vi "Send Value Update.vi"(8 "error in (no error)":errorcluster, 9 "Value":variant, 10 "Datum Name":string, 11 "IViewModel in":refnum<class "IViewModel.lvclass">) -> (0 "error out":errorcluster)   [LabVIEW 2018, in "MVA Framework.lvlib" / "IViewModel.lvlib" / "IViewModel.lvclass"]
doc: "发送值更新"
uses:
  IViewModel.lvclass
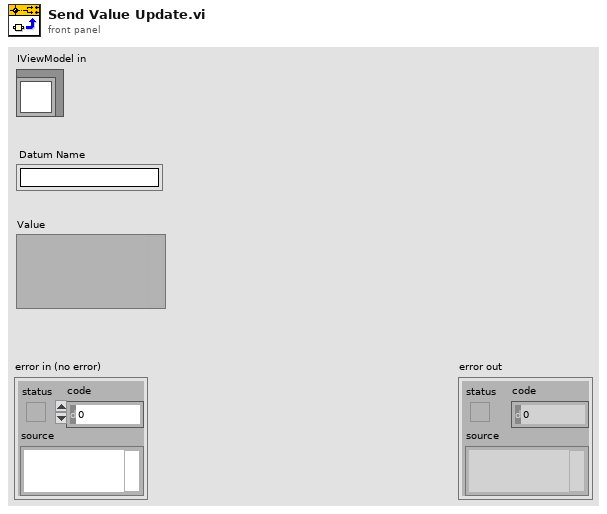
[diagram p1: front panel]
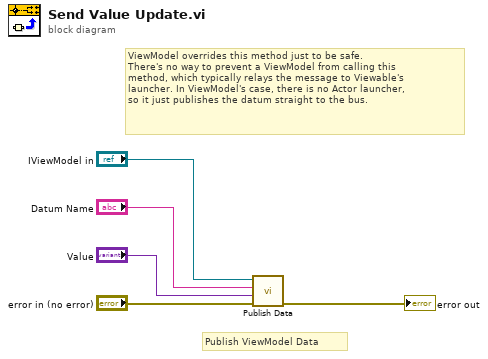
[diagram p0: block diagram]
diagram:
  # "ViewModel overrides this method just to be safe.\nThere's no way to prevent a ViewModel from calling this\nmethod, which typically relays the message to Viewable's\nlauncher. In ViewModel's case, there is no Actor launcher,\nso it just publishes the datum straight to the bus."
  # "Publish ViewModel Data"
  n1 = call "Publish Data.vi"("error in (no error)"="error in (no error)", "Data to Publish"="Value", "Datum Name"="Datum Name", "IViewModel In"="IViewModel in") -> ("error out"=→"error out":errorcluster)  [unwired: 6 in, 1 out]
